vi "Remove Channel.vi"(8 "error in (no error)":errorcluster, 10 "DIO_CFG":refnum<class "DIO-Configuration.lvclass">, 11 "UI Template in":refnum<class "DIO_Panel.lvclass">) -> (0 "error out":errorcluster, 3 "UI Template out":refnum<class "DIO_Panel.lvclass">)   [LabVIEW 2021, in "Simulator-Channel.lvlib" / "DIO_Panel.lvlib" / "DIO_Panel.lvclass"]
uses:
  DIO_Panel.lvclass
  C:/Program Files/National Instruments/LabVIEW 2021/vi.lib/ActorFramework/Actor/Actor.lvclass
  Dependencies/DIO-Channel.lvlibp/Channels/DIO-Channel/DIO-Configuration_class/DIO-Configuration.lvclass
  C:/Users/averna/Documents/LV Gym DEMO/Factory Pattern/Channels/Dependencies/Channel.lvlibp/Channel/Configuration_class/Configuration.lvclass
  DIO_Panel.lvclass/DIO_Panel.ctl
  tdef/info.ctl
  <vilib>/ActorFramework/Actor/Actor.lvclass/Actor.ctl
  <vilib>/ActorFramework/Message Enqueuer/Message Enqueuer.lvclass/Message Enqueuer.ctl
  <vilib>/ActorFramework/Message Enqueuer/Init from Existing Queue.vi
  <vilib>/ActorFramework/Message Enqueuer/Enqueue.vi
  <vilib>/ActorFramework/Stop Msg/Stop Msg.lvclass
  C:/Program Files/National Instruments/LabVIEW 2021/vi.lib/ActorFramework/Message/Message.lvclass
  <vilib>/ActorFramework/Message Priority Queue/Priority Enqueue.vi
  <vilib>/ActorFramework/Message Enqueuer/Message Enqueuer.lvclass
  <vilib>/ActorFramework/Actor/Actor.lvclass
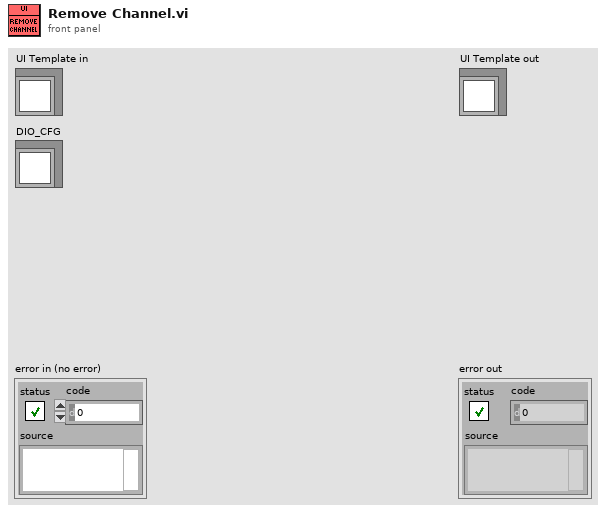
[diagram p1: front panel]
types:
  T1 = typedef "Simulator-Channel.lvlib/DIO_Panel.lvlib/DIO_Panel.lvclass/info.ctl" = cluster{"Name":string, "Boolean":bool}
  T2 = typedef "DIO-Channel.lvlibp/DIO-Configuration.lvclass/Direction.ctl" = enum16{"Input", "Output"}
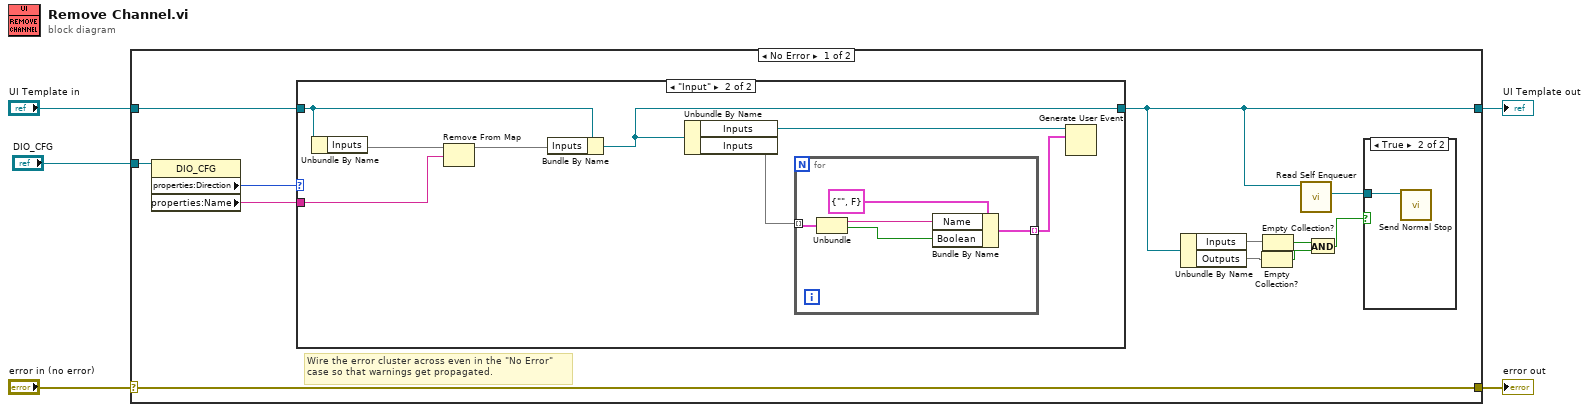
[diagram p0: block diagram]
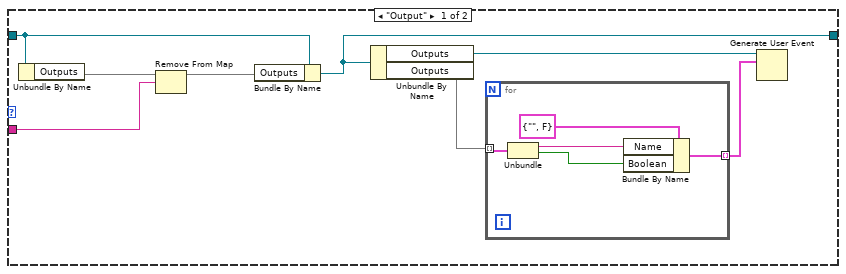
[diagram p3: hidden frame]
diagram:
  n1 = case shown="No Error" "error in (no error)" {
    selector: "error in (no error)" -> [w17 w46]
    tunnel: [w17 w46] -> w4
    tunnel: [w8 w45] -> w2
    tunnel: "UI Template in" -> [w15 w45]
    tunnel: "DIO_CFG" -> [w16 _]
    frame No Error {
      # "Wire the error cluster across even in the \"No Error\"\ncase so that warnings get propagated."
      n2 = property class="DIO_CFG"(reference=w16) -> ("properties:Direction"=w14:T2, "properties:Name"=w13:string)  [unwired: 1 in, 2 out]
      n3 = case shown="\"Input\"" w14 {
        tunnel: [w22 w32] -> w8
        tunnel: w15 -> [w26 w39]
        tunnel: w13 -> [w20 w36]
        frame "Output" {
          n4 = Unbundle By Name(w26) -> ("Outputs"=w21:map{string, bool})
          n5 = Remove From Map(10:w20, 11:w21) -> (3:w19:map{string, bool})  [unwired: 2 out]
          n6 = Bundle By Name(cluster=w26, "Outputs"=w19) -> (w22:refnum<class "DIO_Panel.lvclass">)
          n7 = Unbundle By Name(w22) -> ("Outputs"=w24:refnum<user-event>, "Outputs"=w25:map{string, bool})
          n8 = for {
            tunnel: w25 -> [w31] mode=indexing
            tunnel: [w27] -> w23 mode=indexing
            n9 = Unbundle(w31) -> (w29:string, "Boolean"=w28:bool)
            n10 = Bundle By Name(cluster=T1 {"Name"="", "Boolean"=FALSE} ("Info"), "Name"=w29, "Boolean"=w28) -> (w27:T1)
          }
          n11 = Generate User Event(user event=w24, event data cluster=w23) -> ()  [unwired: 2 in, 2 out]
        }
        frame "Input" {
          n12 = Unbundle By Name(w39) -> ("Inputs"=w38:map{string, bool})
          n13 = Remove From Map(10:w36, 11:w38) -> (3:w37:map{string, bool})  [unwired: 2 out]
          n14 = Bundle By Name(cluster=w39, "Inputs"=w37) -> (w32:refnum<class "DIO_Panel.lvclass">)
          n15 = Unbundle By Name(w32) -> ("Inputs"=w34:refnum<user-event>, "Inputs"=w35:map{string, bool})
          n16 = for {
            tunnel: w35 -> [w44] mode=indexing
            tunnel: [w40] -> w33 mode=indexing
            n17 = Unbundle(w44) -> (w42:string, "Boolean"=w41:bool)
            n18 = Bundle By Name(cluster=T1 {"Name"="", "Boolean"=FALSE} ("Info"), "Name"=w42, "Boolean"=w41) -> (w40:T1)
          }
          n19 = Generate User Event(user event=w34, event data cluster=w33) -> ()  [unwired: 2 in, 2 out]
        }
      }
      n20 = Unbundle By Name(w8) -> ("Inputs"=w12:map{string, bool}, "Outputs"=w11:map{string, bool})
      n21 = Empty Collection?(1:w11) -> (0:w9:bool)
      n22 = Empty Collection?(1:w12) -> (0:w10:bool)
      n23 = call <vilib>:"Read Self Enqueuer.vi"("Actor"=w8) -> ("Self Enqueuer"=w7:refnum<class "Message Enqueuer.lvclass">)  [unwired: 10 in]
      n24 = And(x=w10, y=w9) -> (x .and. y?=w6:bool)
      n25 = case shown="True" w6 {
        tunnel: w7 -> [_ w18]
        frame False {
        }
        frame True {
          n26 = call <vilib>:"Send Normal Stop.vi"("Message Enqueuer"=w18) -> ()  [unwired: 10 in, 1 out]
        }
      }
    }
    frame Error {
    }
  }
  "error out" <- w4
  "UI Template out" <- w2
